vi "TopLevel.vi"(8 "error in (no error)":errorcluster) -> (0 "error out":errorcluster)   [LabVIEW 2020]
uses:
  classes/Test Suite/Test Suite.lvclass
panel:
  out "Test Report File Contents":string
  out "deleted successfully?":bool
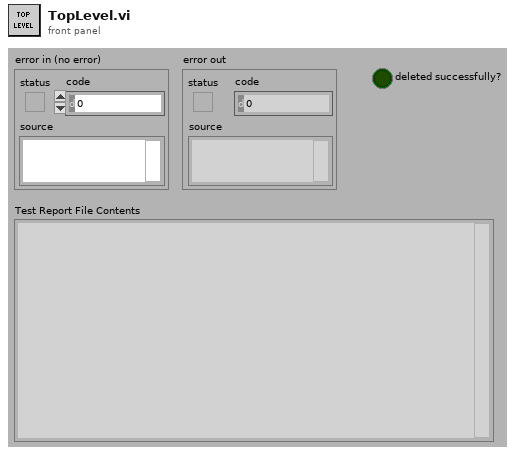
[diagram p1: front panel]
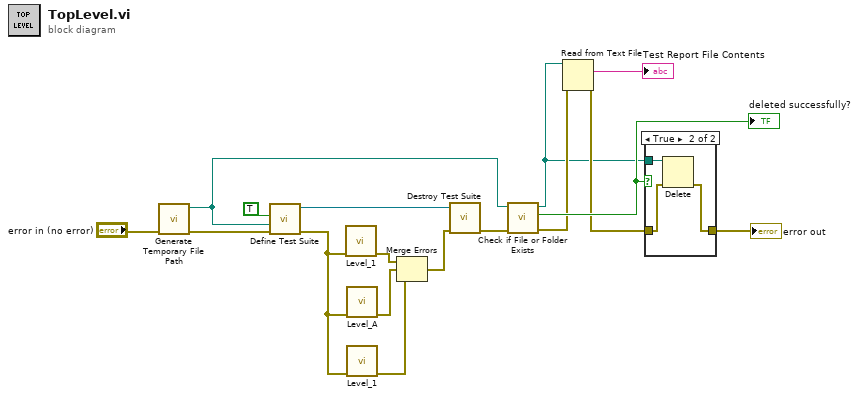
[diagram p0: block diagram]
diagram:
  n1 = call <vilib>:"Generate Temporary File Path.vi"("error in (no error)"="error in (no error)") -> ("error out"=w13:errorcluster, "Unique Temporary File Path"=w11:path)  [unwired: 9 in]
  n2 = call "Define Test Suite.vi"("error in (no error)"=w13, "Report Path"=w11, "Interactive"=TRUE) -> ("error out"=w2:errorcluster, "Test Suite"=w15:refnum<class "Test Suite.lvclass">)  [unwired: 6 in, 1 out]
  n3 = call "Level_1.vi"("error in (no error)"=w2) -> ("error out"=w17:errorcluster)  [unwired: 10 in]
  n4 = call "Level_A.vi"("error in (no error)"=w2) -> ("error out"=w16:errorcluster)  [unwired: 10 in]
  n5 = call "Level_1.vi"("error in (no error)"=w2) -> ("error out"=w1:errorcluster)  [unwired: 10 in]
  n6 = Merge Errors(w17, w16, w1) -> (w3:errorcluster)
  n7 = call-dynamic "Destroy Test Suite.vi"("error in (no error)"=w3, "Test Suite in"=w15) -> ("error out"=w12:errorcluster)  [unwired: 8 in, 1 out]
  n8 = call <vilib>:"Check if File or Folder Exists.vi"("error in (no error)"=w12, "path"=w11) -> ("error out"=w9:errorcluster, "file or folder exists?"=w10:bool, "dup path"=w6:path)  [unwired: 7 in]
  "deleted successfully?" <- w10
  n9 = Read from Text File(file (use dialog)=w6, error in=w9) -> (text=→"Test Report File Contents":string, error out=w8:errorcluster)  [unwired: 2 in, 2 out]
  n10 = case shown="True" w10 {
    tunnel: w6 -> [_ w21]
    tunnel: w8 -> [w18 w20]
    tunnel: [w18 w19] -> w5
    frame False {
    }
    frame True {
      n11 = Delete(path (use dialog)=w21, error in=w20) -> (error out=w19:errorcluster)  [unwired: 3 in, 2 out]
    }
  }
  "error out" <- w5
